vi "Exo_structure_resultat_string.vi"() -> ()   [LabVIEW 2012]
panel:
  in  "Bouton":bool
  out "String":string="resultat positif ou nul "
  out "x-y":dbl
  in  "y":dbl
  in  "x":dbl
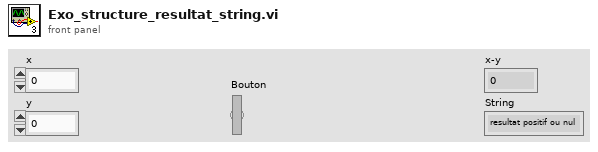
[diagram p1: front panel]
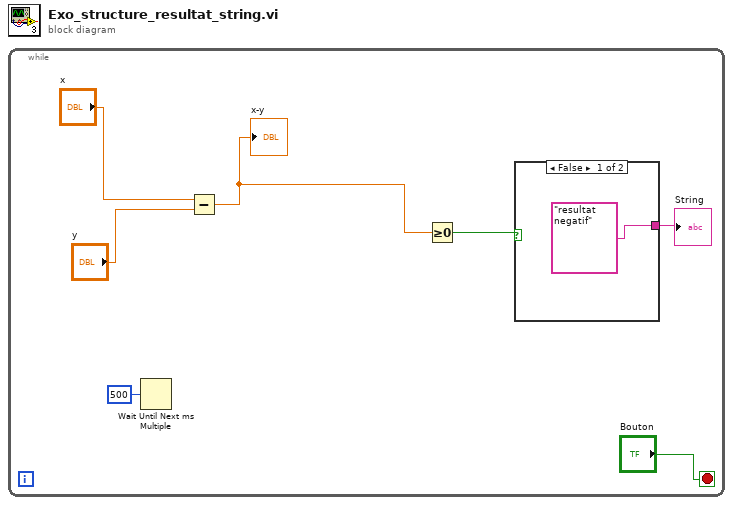
[diagram p0: block diagram]
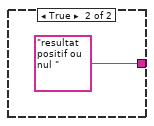
[diagram p2: hidden frame]
diagram:
  n1 = while {
    stop <- "Bouton" stop-if-true
    n2 = Wait Until Next ms Multiple(millisecond multiple=u32 500) -> ()  [unwired: 1 out]
    n3 = Subtract(x="x", y="y") -> (x-y=w5:dbl)
    "x-y" <- w5
    n4 = Greater Or Equal To 0?(x=w5) -> (x >= 0?=w4:bool)
    n5 = case shown="False" w4 {
      tunnel: ["resultat negatif" "resultat positif ou nul "] -> w3
      frame False {
      }
      frame True {
      }
    }
    "String" <- w3
  }
